vi "Construct Path Component.vi"(7 "Strip lead \"/\" (F)":bool, 11 "Segments":string[](array[string])) -> (3 "path":string)   [LabVIEW 2013, in "openURI.lvlib"]
uses:
  openURI.lvlib
  components/path/URI-Component.Path.lvclass
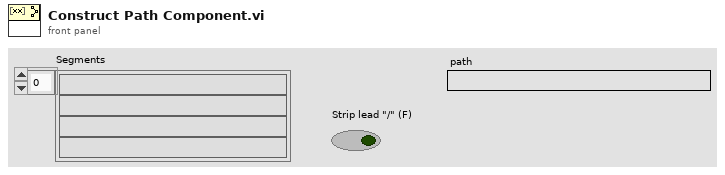
[diagram p1: front panel]
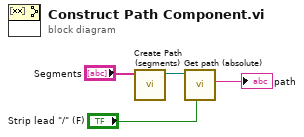
[diagram p0: block diagram]
diagram:
  n1 = call "Create Path (segments).vi"("Segments"="Segments") -> ("URI-Component.Path"=w4:refnum<class "URI-Component.Path.lvclass">)  [unwired: 8 in, 2 out]
  n2 = call "Get path (absolute).vi"("Strip lead \"/\" (F)"="Strip lead \"/\" (F)", "URI-Component.Path in"=w4) -> ("path-component"=→"path":string)  [unwired: 7 in, 2 out]
